vi "Measurement Logic.vi"() -> ()   [LabVIEW 2022 SP3, in "Single Tone_Class D Amplifier.lvlib"]
uses:
  Single Tone_Class D Amplifier.lvlib
  Measurement Results.ctl
  shared/controls/units - snr.ctl
  shared/controls/audio controls.lvlib
  shared/controls/units - ratio.ctl
  shared/controls/units settings.ctl
  shared/controls/weighting filter.ctl
  shared/controls/highpass filter.ctl
  shared/controls/lowpass filter.ctl
  shared/controls/audio filter settings.ctl
  shared/controls/single tone audio measurement settings.ctl
  <vilib>/Waveform/WDTOps.llb/WDT Get Waveform Subset DBL.vi
  <vilib>/DAQmx/read.llb/DAQmx Read (Analog 1D Wfm NChan NSamp).vi
  <vilib>/DAQmx/configure/timing.llb/DAQmx Timing (Sample Clock).vi
  <vilib>/DAQmx/create/channels.llb/DAQmx Create Channel (AI-Voltage-Basic).vi
  shared/digital serial api/Digital Serial.lvclass
  shared/digital serial gen settings/digital audio protocol controls.lvlib
  Measurement Configuration.ctl
  shared/controls/digital output level units.ctl
  shared/controls/single tone audio measurements.ctl
  <vilib>/Plug-In SDKs/Measurements/Measure Call Context/Measure Call Context.lvclass
panel:
  out "names out":string[](array[string])
  out "results":T1[](array[typedef])
  out "Spectrum":cluster{"x0":dbl, "dx":dbl, "magnitude":dbl[]}[](graph)
  out "Waveform Graph":waveform(dbl)[](graph)=[{"t0"=timestamp(3785336549.595634 s since 1904-01-01), "dt"=1.9531249997269942e-05, "Y"=array[12800 elements], "attributes"=variant("NI_ChannelName"=variant(string "PXI1Slot4/ai0"), "NI_UnitDescription"=variant(string "Volts"))}]
  out "measure call context out":refnum<class "Measure Call Context.lvclass">
  in  "measure call context in":refnum<class "Measure Call Context.lvclass">
  out "measurement results":T2={"channel names"=[], "frequency (Hz)"=[], "amplitude (Vrms)"=[], "amplitude (dBFS)"=[], "phase (deg)"=[], "SNR"=[], "THD+N"=[], "THD"=[], "dynamic range (dB)"=[], "gain"=[], "SFDR (dBc)"=[], "output power (W)"=[], "wfm - t0"=0.0, "wfm - dt"=1.9531249997269942e-05, "wfm - data"=array[12800 elements], "fft - f0"=0.0, "fft - df"=4.000000000559116, "fft - data"=array[6400 elements]}
  in  "measurement configuration":T3={"digital serial cfg file"="", "digital channel list"="7821\\PCMo 8", "master clock channel list"="7821\\PCMo 0", "signal frequency"=1000.0, "output level"=1.0, "output level units"=enum."% FS", "output range (pk-pk)"=15.0, "load impedance"=4.0, "signal phase"=0.0, "acq sampling rate"=51200.0, "min measurement cycles"=20, "min measurement time (s)"=0.1, "min settling cycles"=0, "min settling time (s)"=0.005, "acq channel"="PXI1Slot4/ai0", "band start"=20.0, "band stop"=20000.0, "weighting filter"=enum."Linear", "lowpass filter"=enum."No filter", "highpass filter"=enum."DC", "SNR units"=enum."dB", "THD+N units"=enum."dB", "THD units"=enum."dB", "gain units"=enum."dB"} {"acq sampling rate" format="%#_6p"}
  out "error out":errorcluster
  in  "error in":errorcluster
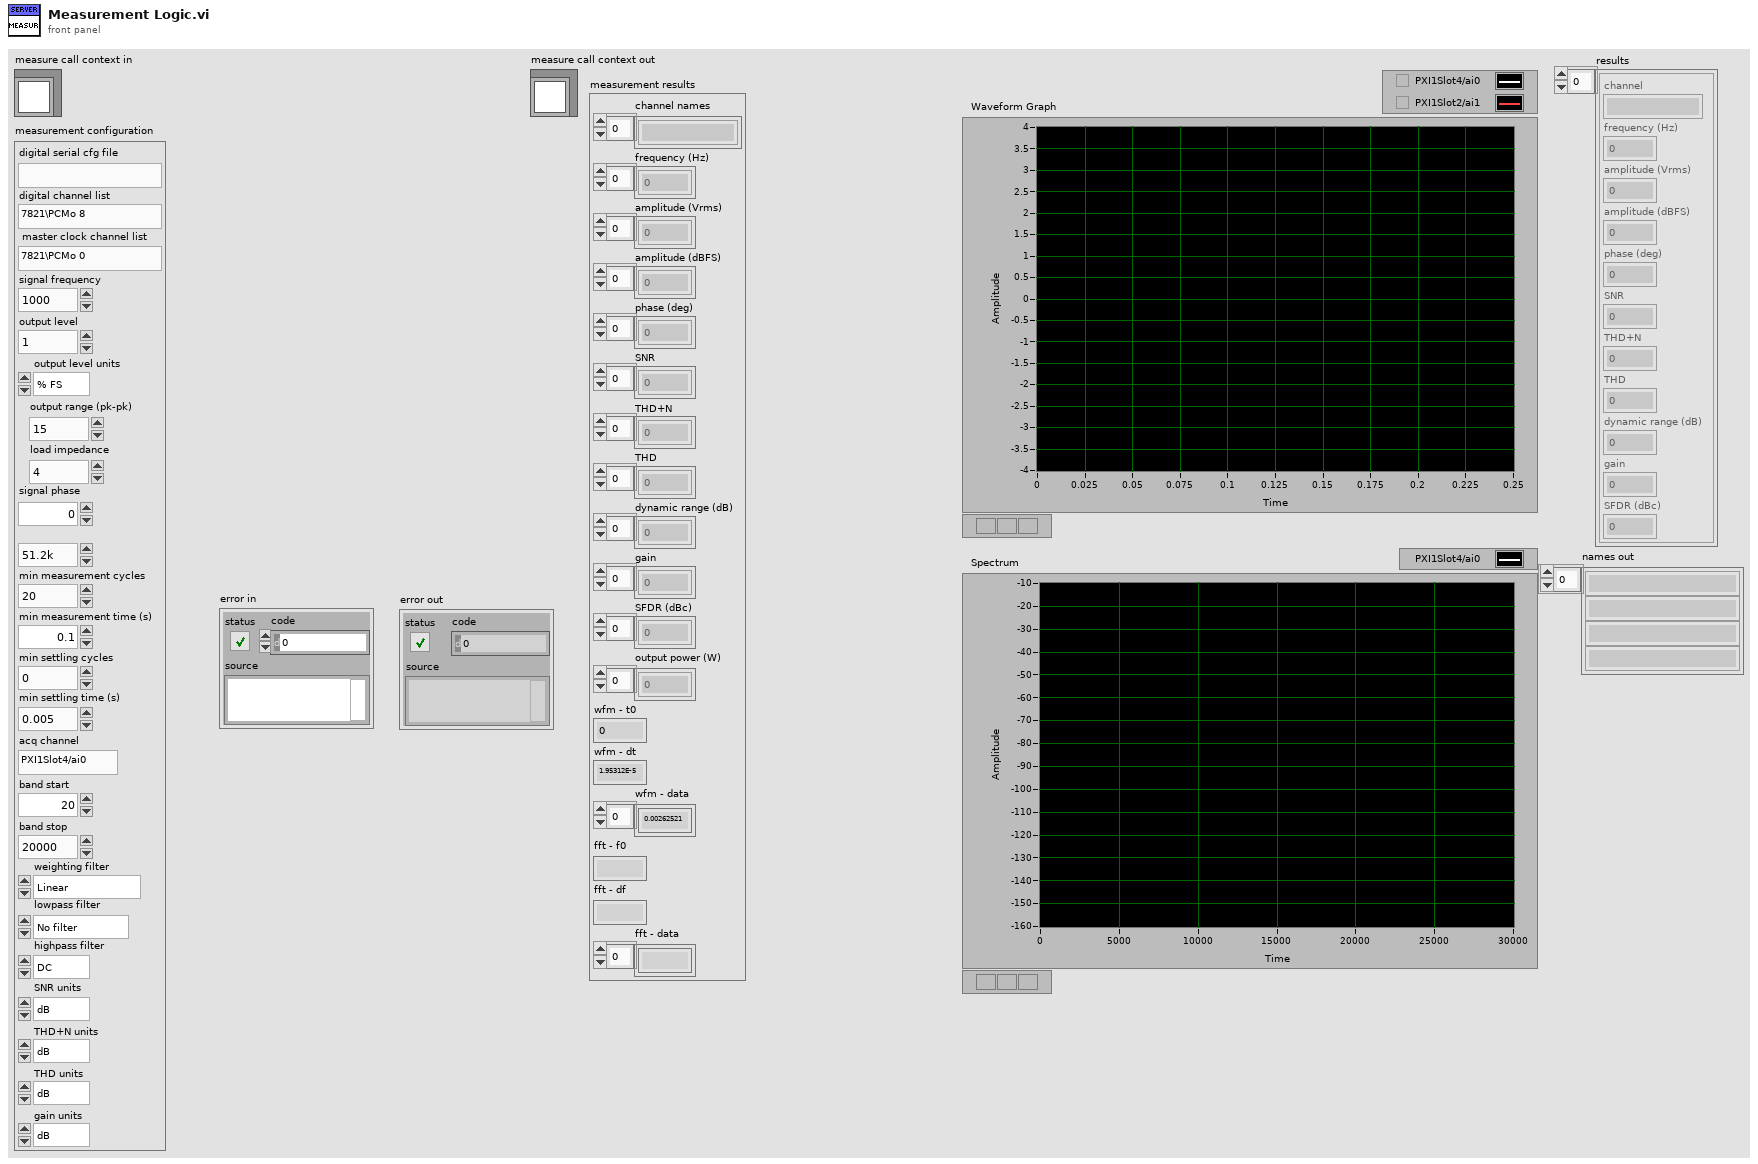
[diagram p1: front panel]
types:
  T1 = typedef "audio controls.lvlib/single tone audio measurements.ctl" = cluster{"channel":string, "frequency (Hz)":dbl, "amplitude (Vrms)":dbl, "amplitude (dBFS)":dbl, "phase (deg)":dbl, "SNR":dbl, "THD+N":dbl, "THD":dbl, "dynamic range (dB)":dbl, "gain":dbl, "SFDR (dBc)":dbl}
  T2 = typedef "Single Tone_Class D Amplifier.lvlib/Measurement Results.ctl" = cluster{"channel names":string[], "frequency (Hz)":dbl[], "amplitude (Vrms)":dbl[], "amplitude (dBFS)":dbl[], "phase (deg)":dbl[], "SNR":dbl[], "THD+N":dbl[], "THD":dbl[], "dynamic range (dB)":dbl[], "gain":dbl[], "SFDR (dBc)":dbl[], "output power (W)":dbl[], "wfm - t0":dbl, "wfm - dt":dbl, "wfm - data":dbl[], "fft - f0":dbl, "fft - df":dbl, "fft - data":dbl[]}
  T3 = typedef "Single Tone_Class D Amplifier.lvlib/Measurement Configuration.ctl" = cluster{"digital serial cfg file":string, "digital channel list":string, "master clock channel list":string, "signal frequency":dbl, "output level":dbl, "output level units":T4, "output range (pk-pk)":dbl, "load impedance":dbl, "signal phase":dbl, "acq sampling rate":dbl, "min measurement cycles":u32, "min measurement time (s)":dbl, "min settling cycles":u32, "min settling time (s)":dbl, "acq channel":string, "band start":dbl, "band stop":dbl, "weighting filter":T5, "lowpass filter":T6, "highpass filter":T7, "SNR units":T8, "THD+N units":T9, "THD units":T9, "gain units":T9}
  T4 = typedef "audio controls.lvlib/digital output level units.ctl" = enum32{"% FS", "dBFS", "V"}
  T5 = typedef "weighting filter.ctl" = enum32{"Linear", "A-weighting", "B-weighting", "C-weighting"}
  T6 = typedef "lowpass filter.ctl" = enum32{"No filter", "AES17 20kHz", "AES17 40kHz"}
  T7 = typedef "highpass filter.ctl" = enum32{"DC", "AC"}
  T8 = typedef "audio controls.lvlib/units - snr.ctl" = enum32{"dB", "x/y"}
  T9 = typedef "audio controls.lvlib/units - ratio.ctl" = enum32{"dB", "%", "x/y"}
  T10 = cluster{"frequency":dbl, "amplitude":dbl, "phase":dbl}
  T11 = typedef "audio controls.lvlib/units settings.ctl" = cluster{"SNR units":T8, "THD+N units":T9, "THD units":T9, "gain units":T9}
  T12 = typedef "audio filter settings.ctl" = cluster{"weighting filter":T5, "highpass filter":T7, "lowpass filter ":T6}
  T13 = typedef "single tone audio measurement settings.ctl" = cluster{"Band start":dbl, "Band stop":dbl, "Amplitude":dbl, "Frequency":dbl, "Full scale range":dbl}
  T14 = typedef "digital serial gen settings.ctl" = cluster{"number of channels":u32, "data justification":T15, "endianness":T16, "channel length":u32, "bit depth":u32, "frame clock rate":dbl, "bit clock edge sync":T17, "master clock rate":dbl, "Logic Level":T18, "frame sync edge for channel 0":T17, "Channel 0 Offset":u32}
  T15 = typedef "PDM Shared.lvlib/PCM Data Justification.ctl" = enum16{"Left Justified", "Right Justified"}
  T16 = typedef "PDM Shared.lvlib/PCM Bit Endianness.ctl" = enum16{"MSB First", "LSB First"}
  T17 = typedef "PDM Shared.lvlib/Digital Edge.ctl" = enum8{"Rising", "Falling"}
  T18 = typedef "PDM Acquisition Class Library.lvlib/DecoderSession.lvclass/Logic Levels.ctl" = enum16{"3.3 V", "1.8 V", "1.2 V"}
  T19 = typedef "AudioGenTypeDefs.lvlib/digital protocol settings.ctl" = cluster{"logic level":T18, "PCM Data Configuration":T20, "bit clock rate":sgl, "master clock rate":sgl, "clock mode":T21, "Frame Sync Clock Control":T22}
  T20 = typedef "PDM Shared.lvlib/PCM Data Format Configuration.ctl" = cluster{"Frame Sync Edge for Channel 0":T17, "Channel Count Per Frame":u8, "Channel Length":u16, "Bit Depth":u8, "Channel 0 Offset":u16, "Endianness":T16, "Data Justification":T15}
  T21 = typedef "PDM Shared.lvlib/clock mode.ctl" = enum16{"divided clock", "DDS"}
  T22 = typedef "PDM Shared.lvlib/PCM Frame Sync Control.ctl" = cluster{"Frame Length":u16, "Frame Sync Pulse Width":u16, "Bit Clock Edge  Sync":T17}
  T23 = cluster{"frequency":dbl, "amplitude":dbl, "phase":dbl}[]
  T24 = typedef "audio controls.lvlib/single tone audio measurements (N chan).ctl" = cluster{"channel names":string[], "frequency (Hz)":dbl[], "amplitude (Vrms)":dbl[], "amplitude (dBFS)":dbl[], "phase (deg)":dbl[], "SNR":dbl[], "THD+N":dbl[], "THD":dbl[], "dynamic range (dB)":dbl[], "gain":dbl[], "SFDR (dBc)":dbl[]}
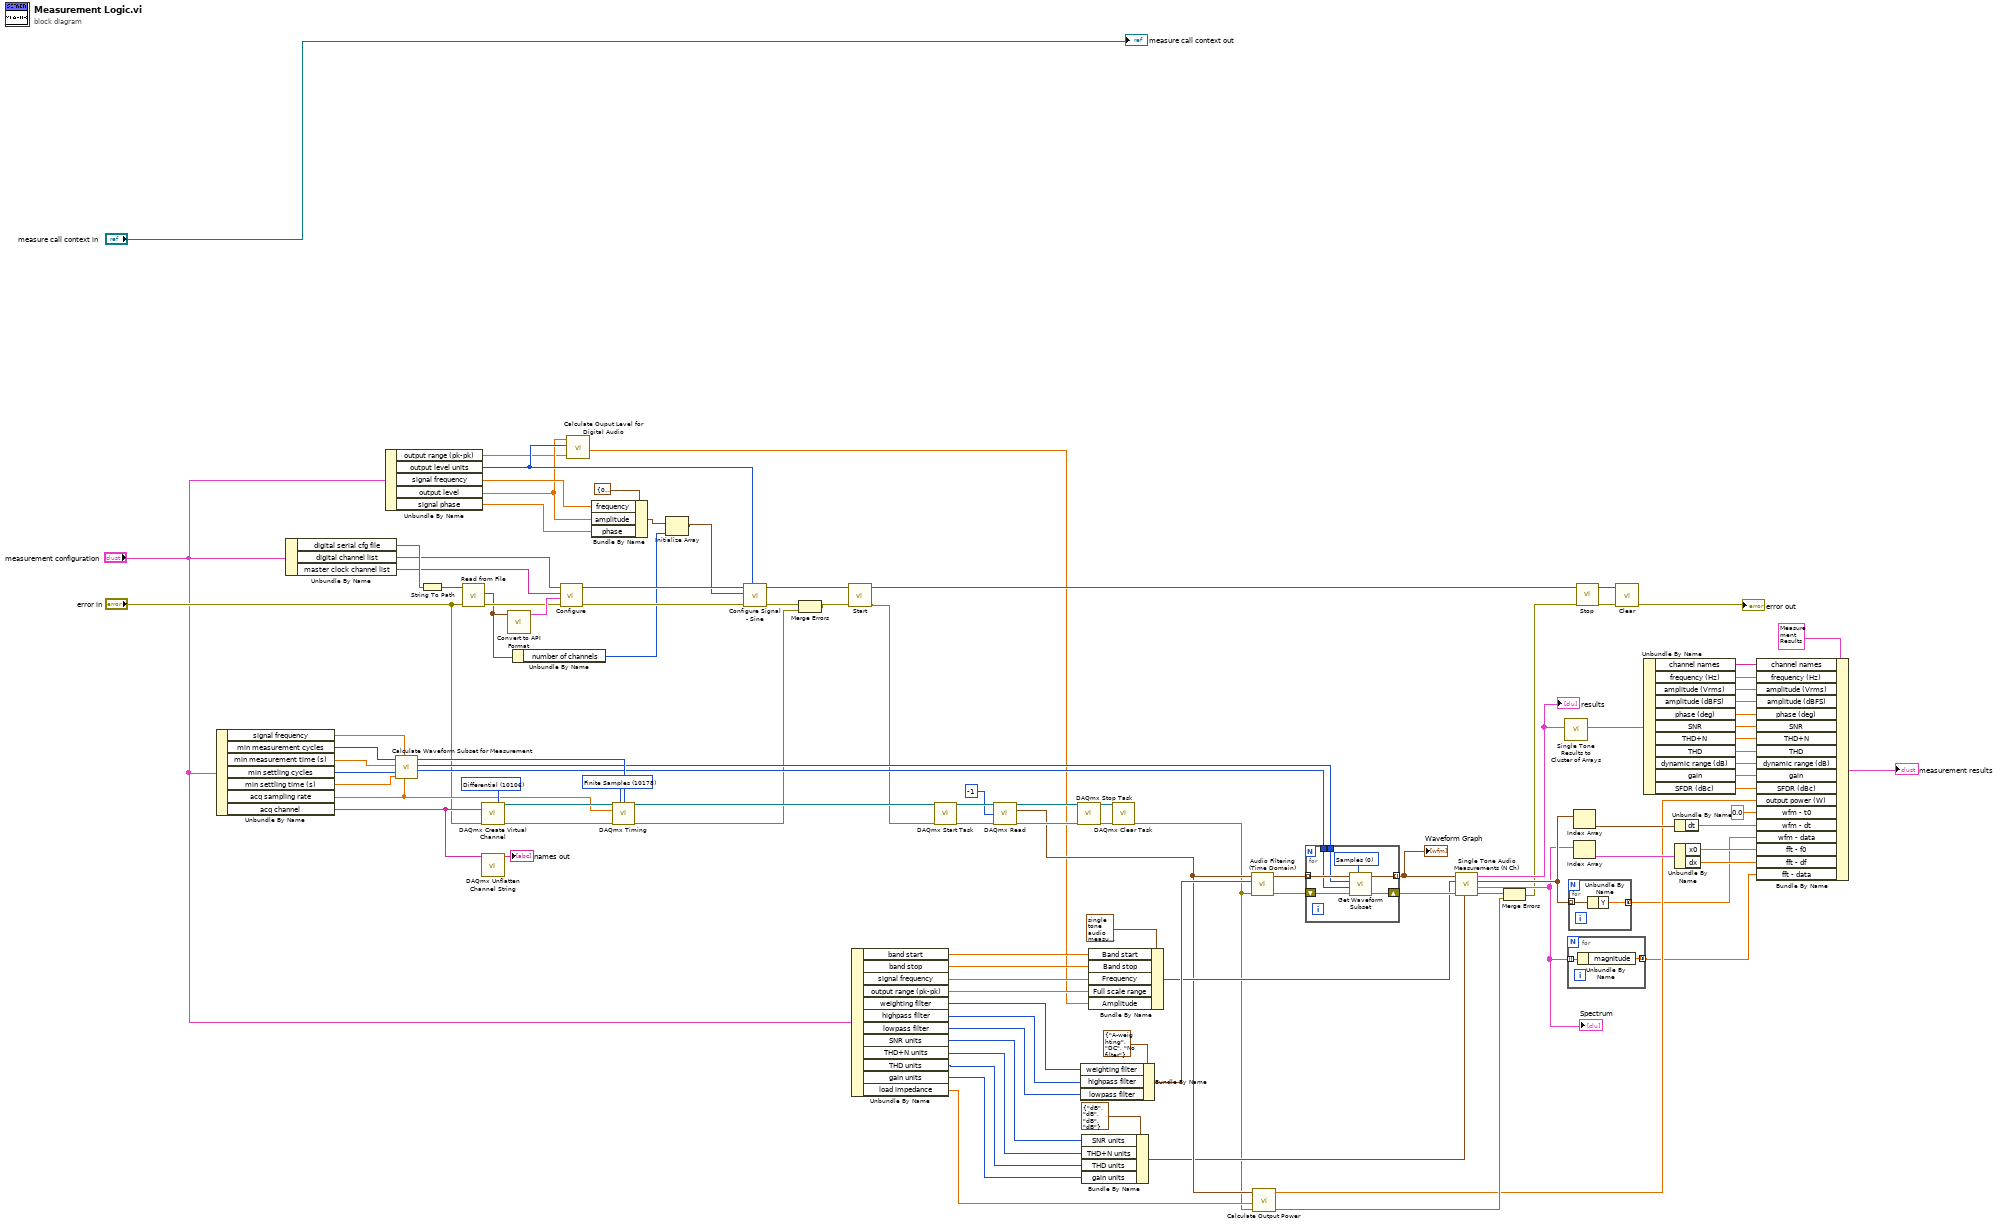
[diagram p0: block diagram]
diagram:
  w92 = 10106 items=["Default"=-1, "RSE"=10083, "NRSE"=10078, "Differential"=10106, "Pseudodifferential"=12529] ("input terminal configuration")
  w97 = 10178 items=["Finite Samples"=10178, "Continuous Samples"=10123, "Hardware Timed Single Point"=12522] ("sample mode")
  n1 = Unbundle By Name("measurement configuration") -> ("signal frequency"=w70:dbl, "min measurement cycles"=w74:u32, "min measurement time (s)"=w73:dbl, "min settling cycles"=w72:u32, "min settling time (s)"=w71:dbl, "acq sampling rate"=w68:dbl, "acq channel"=w53:string)
  n2 = Unbundle By Name("measurement configuration") -> ("digital serial cfg file"=w31:string, "digital channel list"=w27:string, "master clock channel list"=w26:string)
  n3 = Unbundle By Name("measurement configuration") -> ("output range (pk-pk)"=w2:dbl, "output level units"=w4:T4, "signal frequency"=w9:dbl, "output level"=w3:dbl, "signal phase"=w8:dbl)
  n4 = call "Calculate Waveform Subset for Measurement.vi"("sampling rate"=w68, "signal frequency"=w70, "minimum settling duration"=w71, "minimum settling cycles"=w72, "minimum measurement duration"=w73, "minimum measurement cycles"=w74) -> ("duration (samples)"=w65:u32, "start (samples)"=w66:u32, "total acquisition (samples)"=w67:u32)  [unwired: 3 in]
  n5 = String To Path(string=w31) -> (path=w28:path)
  n6 = call "Read from File.vi"("error in (no error)"="error in", "file path"=w28) -> ("error out"=w29:errorcluster, "digital audio protocol settings"=w23:T14)  [unwired: 7 in, 1 out]
  n7 = call-poly <vilib>:"DAQmx Create Virtual Channel.vi"("input terminal configuration"=w92, "physical channels"=w53, "error in"="error in") -> ("task out"=w105:refnum<k21>, "error out"=w106:errorcluster)  [unwired: 11 in]
  n8 = call <vilib>:"DAQmx Unflatten Channel String.vi"("names in"=w53) -> ("names out"=→"names out":string[])  [unwired: 13 in, 1 out]
  n9 = call "Convert to API Format.vi"("digital audio protocol settings"=w23) -> ("digital protocol settings"=w30:T19)  [unwired: 10 in]
  n10 = Unbundle By Name(w23) -> ("number of channels"=w6:u32)
  n11 = call "Configure.vi"("error in (no error)"=w29, "digital protocol settings"=w30, "master clock channel list"=w26, "data channel list"=w27) -> ("error out"=w25:errorcluster, "digital serial task"=w24:refnum<class "Digital Serial.lvclass">)  [unwired: 6 in]
  n12 = call "Calculate Ouput Level for Digital Audio.vi"("output range (pk-pk)"=w2, "digital output level units"=w4, "output level"=w3) -> ("amplitude (pk)"=w1:dbl)  [unwired: 7 in, 1 out]
  n13 = Bundle By Name(cluster=T10 {"frequency"=0.0, "amplitude"=0.0, "phase"=0.0} ("sine wave"), "frequency"=w9, "amplitude"=w3, "phase"=w8) -> (w7:T10)
  n14 = call-poly <vilib>:"DAQmx Timing.vi"("task/channels in"=w105, "sample mode"=w97, "samples per channel"=w67, "rate"=w68, "error in"=w106) -> ("task out"=w98:refnum<k21>, "error out"=w18:errorcluster)  [unwired: 9 in]
  n15 = Initialize Array(w7, w6) -> (w5:T23)
  n16 = call "Configure Signal - Sine.vi"("output level units"=w4, "error in (no error)"=w25, "sine wave properties"=w5, "Digital Serial in"=w24) -> ("error out"=w20:errorcluster, "Digital Serial out"=w19:refnum<class "Digital Serial.lvclass">)  [unwired: 6 in]
  n17 = Merge Errors(w20, w18) -> (w21:errorcluster)
  n18 = call "Start.vi"("error in (no error)"=w21, "Digital Serial in"=w19) -> ("error out"=w17:errorcluster, "Digital Serial out"=w14:refnum<class "Digital Serial.lvclass">)  [unwired: 8 in]
  n19 = Unbundle By Name("measurement configuration") -> ("band start"=w84:dbl, "band stop"=w83:dbl, "signal frequency"=w75:dbl, "output range (pk-pk)"=w76:dbl, "weighting filter"=w81:T5, "highpass filter"=w80:T7, "lowpass filter"=w79:T6, "SNR units"=w61:T8, "THD+N units"=w60:T9, "THD units"=w59:T9, "gain units"=w58:T9, "load impedance"=w62:dbl)
  n20 = call <vilib>:"DAQmx Start Task.vi"("task/channels in"=w98, "error in"=w17) -> ("task out"=w100:refnum<k21>, "error out"=w103:errorcluster)  [unwired: 12 in]
  n21 = call-poly <vilib>:"DAQmx Read.vi"("task/channels in"=w100, "number of samples per channel"=-1, "error in"=w103) -> ("task out"=w99:refnum<k21>, "data"=w69:waveform(dbl)[], "error out"=w102:errorcluster)  [unwired: 10 in]
  n22 = call <vilib>:"DAQmx Stop Task.vi"("task/channels in"=w99, "error in"=w102) -> ("task out"=w104:refnum<k21>, "error out"=w101:errorcluster)  [unwired: 12 in]
  n23 = Bundle By Name(cluster=T12 {"weighting filter"=enum."A-weighting", "highpass filter"=enum."DC", "lowpass filter "=enum."No filter"} ("filter settings"), "weighting filter"=w81, "highpass filter"=w80, "lowpass filter"=w79) -> (w78:T12)
  n24 = Bundle By Name(cluster=T11 {"SNR units"=enum."dB", "THD+N units"=enum."dB", "THD units"=enum."dB", "gain units"=enum."dB"} ("units settings"), "SNR units"=w61, "THD+N units"=w60, "THD units"=w59, "gain units"=w58) -> (w63:T11)
  n25 = Bundle By Name(cluster=T13 {"Band start"=20.0, "Band stop"=20000.0, "Amplitude"=-1.0, "Frequency"=1000.0, "Full scale range"=15.0} ("measurement settings"), "Band start"=w84, "Band stop"=w83, "Frequency"=w75, "Full scale range"=w76, "Amplitude"=w1) -> (w77:T13)
  n26 = call <vilib>:"DAQmx Clear Task.vi"("task in"=w104, "error in"=w101) -> ("error out"=w57:errorcluster)  [unwired: 13 in]
  n27 = call "Audio Filtering (Time Domain).vi"("waveforms"=w69, "filter settings"=w78, "error in"=w57) -> ("time domain"=w88:waveform(dbl)[], "error out"=w89:errorcluster)  [unwired: 6 in]
  n28 = call "Calculate Output Power.vi"("error in (no error)"=w57, "load impedance"=w62, "waveforms"=w69) -> ("error out"=w90:errorcluster, "output power"=w36:dbl[])  [unwired: 7 in]
  n29 = for {
    tunnel: w88 -> [w114] mode=indexing
    tunnel: [w113] -> w56 mode=indexing
    shift-right: [w110] -> w87
    shift-left: w89 -> [w111]
    tunnel: w66 -> [w109]
    tunnel: w65 -> [w108]
    w112 = u16 0 items=["Samples", "Relative Time"] ("start/duration format")
    n30 = call-poly <vilib>:"Get Waveform Subset.vi"("start/duration format"=w112, "error in (no error)"=w111, "duration"=w108, "start samples/time"=w109, "waveform in"=w114) -> ("error out"=w110:errorcluster, "waveform out"=w113:waveform(dbl))  [unwired: 1 in, 2 out]
  }
  "Waveform Graph" <- w56
  n31 = call "Single Tone Audio Measurements (N Ch).vi"("units settings"=w63, "error in"=w87, "measurement settings"=w77, "waveforms"=w56) -> ("error out"=w86:errorcluster, "spectra"=w34:cluster{"x0":dbl, "dx":dbl, "magnitude":dbl[]}[], "waveforms"=w35:waveform(dbl)[], "results"=w49:T1[])  [unwired: 4 in]
  "Spectrum" <- w34
  "results" <- w49
  n32 = Merge Errors(w86, w90) -> (w13:errorcluster)
  n33 = call "Single Tone Results to Cluster of Arrays.vi"("results"=w49) -> ("results (N chan)"=w48:T24)  [unwired: 10 in]
  n34 = for {
    tunnel: w34 -> [w116] mode=indexing
    tunnel: [w115] -> w33 mode=concatenating
    n35 = Unbundle By Name(w116) -> ("magnitude"=w115:dbl[])
  }
  n36 = for {
    tunnel: w35 -> [w118] mode=indexing
    tunnel: [w117] -> w32 mode=concatenating
    n37 = Unbundle By Name(w118) -> ("Y"=w117:dbl[])
  }
  n38 = Index Array(array=w35) -> (element=w55:waveform(dbl))  [unwired: 1 in]
  n39 = Index Array(array=w34) -> (element=w54:cluster{"x0":dbl, "dx":dbl, "magnitude":dbl[]})  [unwired: 1 in]
  n40 = call "Stop.vi"("error in (no error)"=w13, "Digital Serial in"=w14) -> ("error out"=w16:errorcluster, "Digital Serial out"=w15:refnum<class "Digital Serial.lvclass">)  [unwired: 8 in]
  n41 = call "Clear.vi"("error in (no error)"=w16, "Digital Serial in"=w15) -> ("error out"=→"error out":errorcluster)  [unwired: 9 in]
  n42 = Unbundle By Name(w48) -> ("channel names"=w47:string[], "frequency (Hz)"=w46:dbl[], "amplitude (Vrms)"=w45:dbl[], "amplitude (dBFS)"=w44:dbl[], "phase (deg)"=w43:dbl[], "SNR"=w42:dbl[], "THD+N"=w41:dbl[], "THD"=w40:dbl[], "dynamic range (dB)"=w39:dbl[], "gain"=w38:dbl[], "SFDR (dBc)"=w37:dbl[])
  n43 = Unbundle By Name(w55) -> ("dt"=w95:dbl)
  n44 = Unbundle By Name(w54) -> ("x0"=w94:dbl, "dx"=w93:dbl)
  n45 = Bundle By Name(cluster=T2 {"channel names"=[], "frequency (Hz)"=[], "amplitude (Vrms)"=[], "amplitude (dBFS)"=[], "phase (deg)"=[], "SNR"=[], "THD+N"=[], "THD"=[], "dynamic range (dB)"=[], "gain"=[], "SFDR (dBc)"=[], "output power (W)"=[], "wfm - t0"=0.0, "wfm - dt"=0.0, "wfm - data"=[], "fft - f0"=0.0, "fft - df"=0.0, "fft - data"=[]} ("Measurement Results"), "channel names"=w47, "frequency (Hz)"=w46, "amplitude (Vrms)"=w45, "amplitude (dBFS)"=w44, "phase (deg)"=w43, "SNR"=w42, "THD+N"=w41, "THD"=w40, "dynamic range (dB)"=w39, "gain"=w38, "SFDR (dBc)"=w37, "output power (W)"=w36, "wfm - t0"=0.0, "wfm - dt"=w95, "wfm - data"=w32, "fft - f0"=w94, "fft - df"=w93, "fft - data"=w33) -> (→"measurement results":T2)
  "measure call context out" <- "measure call context in"
